vi "Host Image Acquisition Loop.vi"(8 "error in":errorcluster) -> (0 "error out":errorcluster)   [LabVIEW 2013]
doc: "Loop handles the image acquisition communication to FPGA.\nInitialize - Queues up the intialize states\n\nExit"
uses:
  Host Image Acquisition Module Enum.ctl
  Message Passing/MsgQ Loops enum.ctl
  File IO/Save Image Module Enum.ctl
  Image Acquisition Settings FG Enum.ctl
  System Status/Status FG Enum.ctl
  Globals/Simulation Settings Global.vi
  Common/State Machines/State Machine Lib.lvlib
  Message Passing/Main MsgQ.lvlib
panel:
  out "State":string
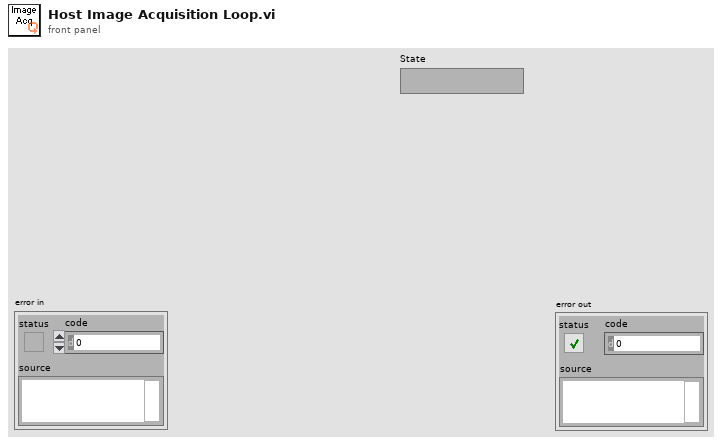
[diagram p1: front panel]
types:
  T1 = typedef "State Machine Lib.lvlib/STATE cluster.ctl" = cluster{"State":string, "Parameters":variant}
  T2 = typedef "Host Image Acquisition Module Enum.ctl" = enum16{"Open FPGA", "Initialize DMA FIFO", "Load Sim Images", "Initialize Acquisition", "Update Sector Parameters", "Start Acquisition", "Aquire Image", "Read Averages", "Cancel Acquisition", "Close FPGA"}
  T3 = typedef "Main MsgQ.lvlib/MsgQ Loops enum.ctl" = enum16{"User Interface", "Image Acq"}
  T4 = typedef "Save Image Module Enum.ctl" = enum16{"Create File", "Write to File", "Status", "Close File"}
  T5 = typedef "Image Acquisition Settings FG Enum.ctl" = enum16{"Read", "Write"}
  T6 = typedef "Status FG Enum.ctl" = enum16{"Reset", "Read", "Write"}
  T7 = typedef "Simulation Settings Cluster.ctl" = cluster{"Sim Enabled?":bool, "Sim Path":path}
  T8 = typedef "Acquisition Settings Cluster.ctl" = cluster{"Image Width":u32, "Image Height":u32, "Frames To Acquire":u32, "Signal Mapping":enum8{"Standard", "Basler 10-tap", "Vosskühler 10-tap"}, "DMA Buffer Size\n(In Images)":u32}
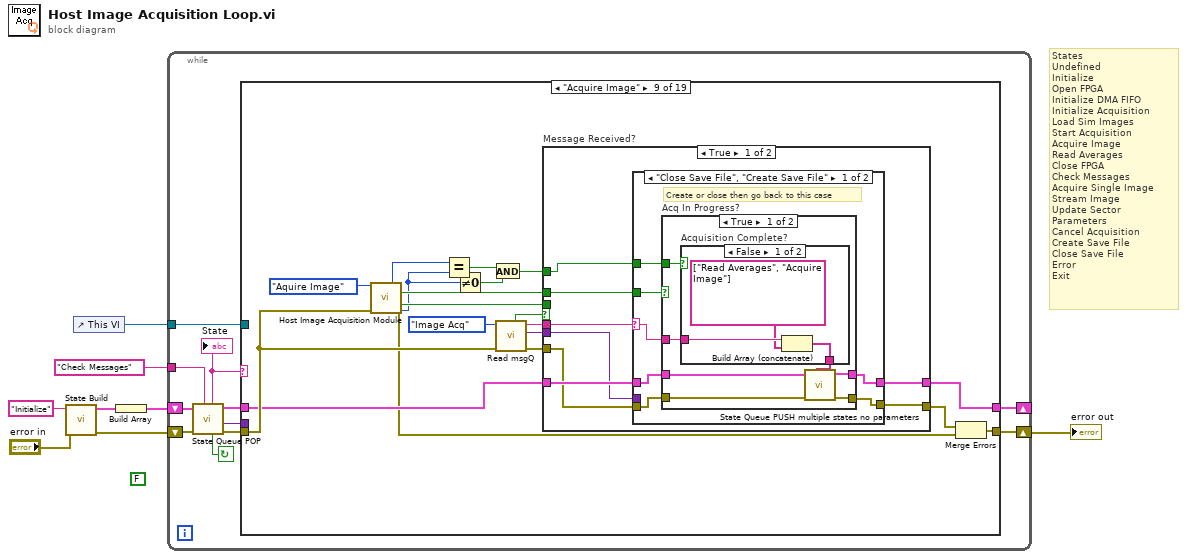
[diagram p0: block diagram]
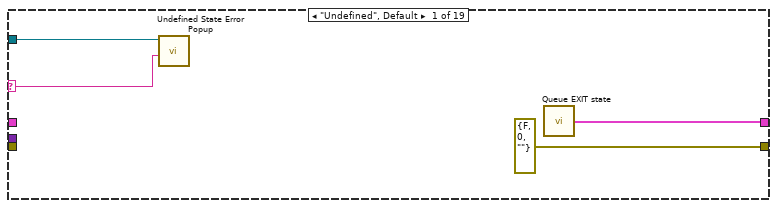
[diagram p2: hidden frame]
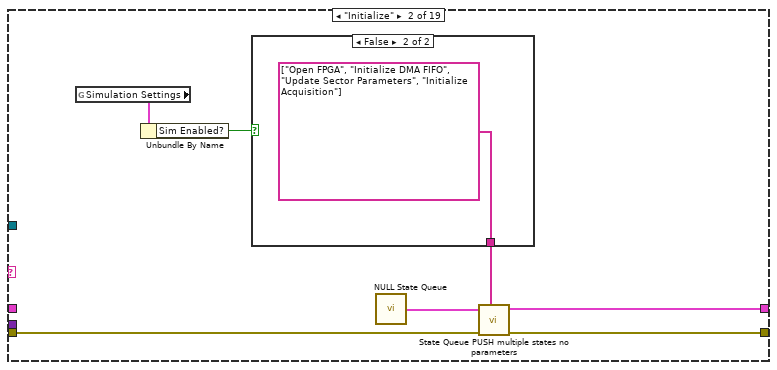
[diagram p3: hidden frame]
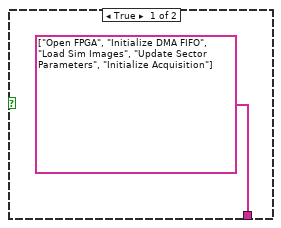
[diagram p4: hidden frame]
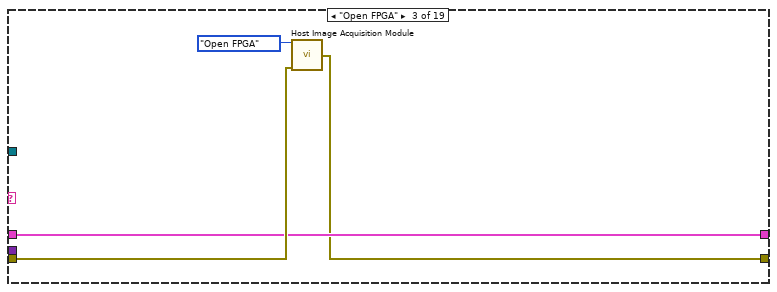
[diagram p5: hidden frame]
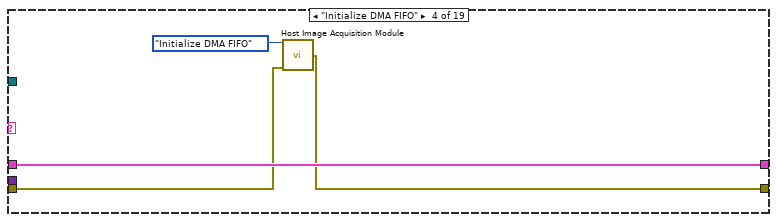
[diagram p6: hidden frame]
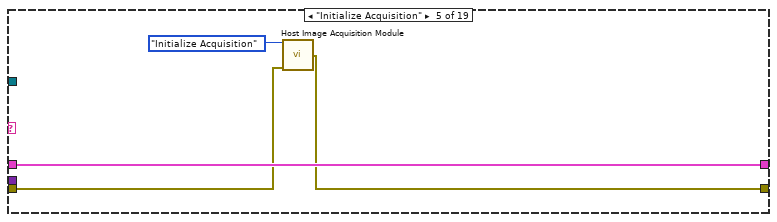
[diagram p7: hidden frame]
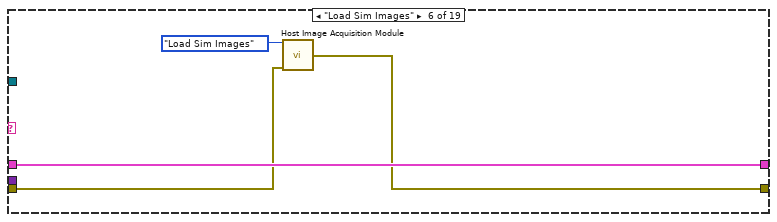
[diagram p8: hidden frame]
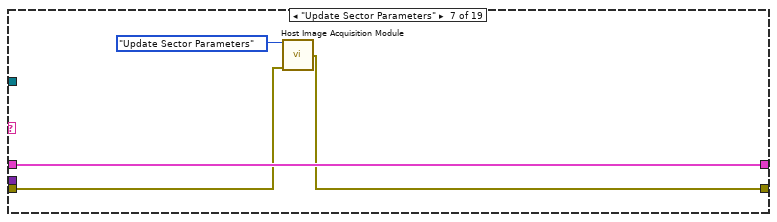
[diagram p9: hidden frame]
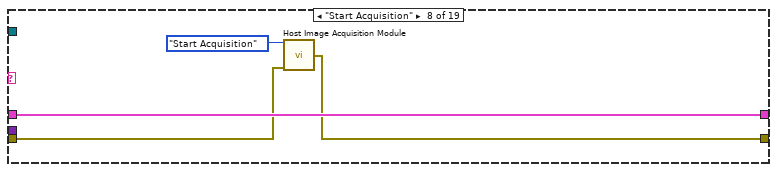
[diagram p10: hidden frame]
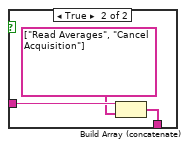
[diagram p11: hidden frame]
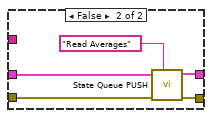
[diagram p12: hidden frame]
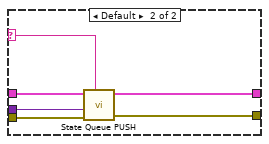
[diagram p13: hidden frame]
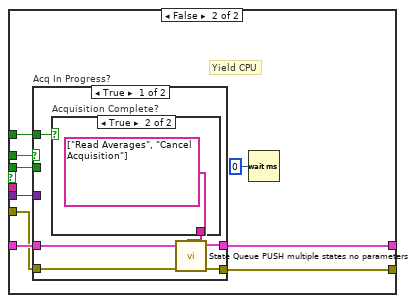
[diagram p14: hidden frame]
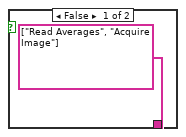
[diagram p15: hidden frame]
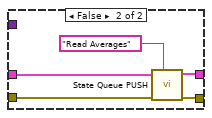
[diagram p16: hidden frame]
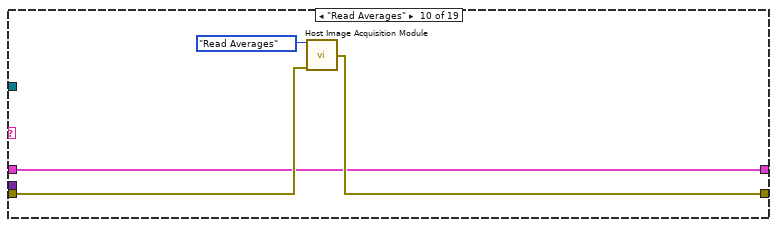
[diagram p17: hidden frame]
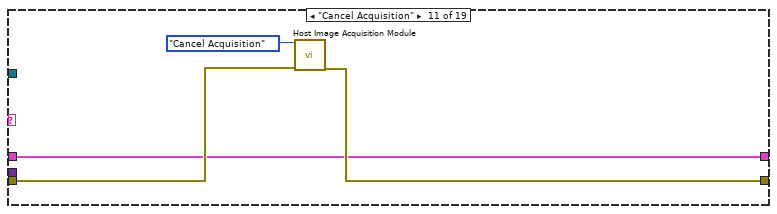
[diagram p18: hidden frame]
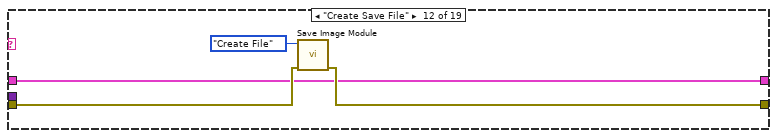
[diagram p19: hidden frame]
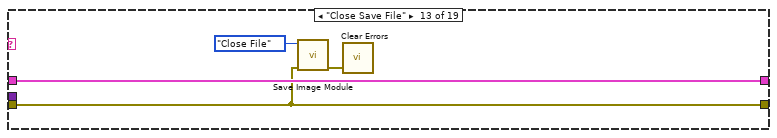
[diagram p20: hidden frame]
diagram:
  (unwired) FALSE
  # "States\nUndefined\nInitialize\nOpen FPGA\nInitialize DMA FIFO\nInitialize Acquisition\nLoad Sim Images\nStart Acquisition\nAcquire Image\nRead Averages\nClose FPGA\nCheck Messages\nAcquire Single Image\nStream Image\nUpdate Sector Parameters\nCancel Acquisition\nCreate Save File\nClose Save File\nError\nExit"
  n1 = call "State Build.vi"("error in (no error)"="error in", "State"="Initialize") -> ("error out"=w4:errorcluster, "State Out"=w6:T1)  [unwired: 8 in]
  n2 = control-ref of="This VI"() -> (w1:refnum<vi>)
  n3 = Build Array(w6) -> (w5:T1[])
  n4 = while {
    shift-right: [w12] -> _
    shift-left: w5 -> [w19]
    shift-right: [w11] -> w2
    shift-left: w4 -> [w18]
    tunnel: "Check Messages" ("Default state") -> [w16]
    tunnel: w1 -> [w10]
    stop <- w17 continue-if-true
    n5 = call "State Queue POP.vi"("Default state"=w16, "error in (no error)"=w18, "State que in"=w19) -> ("error out"=w13:errorcluster, "Parameters"=w9:variant, "State que out"=w14:T1[], "Not Exit?"=w17:bool, "State case out"=w15:string)  [unwired: 4 in]
    "State" <- w15
    n6 = case shown="\"Acquire Image\"" w15 {
      selector: w15 -> [w22 _ _ _ _ _ _ _ _ _ _ _ _ _ _ _ _ _ _]
      tunnel: w14 -> [_ _ w34 w40 w44 w48 w52 w56 w73 w137 w141 w145 w151 w156 w163 w178 w199 w219 w226]
      tunnel: w13 -> [_ w30 w35 w39 w43 w47 w51 w55 w74 w139 w143 w147 w149 w155 w165 w185 w189 w222 w225]
      tunnel: [w21 w27 w34 w40 w44 w48 w52 w56 w72 w137 w141 w145 w151 w156 w162 w176 w194 w219 w226] -> w12
      tunnel: [errorcluster {"status"=FALSE, "code"=0, "source"=""} ("error out") w26 w33 w38 w42 w45 w50 w54 w70 w138 w142 w146 w149 w154 w161 w175 w192 w220 w225] -> w11
      tunnel: w10 -> [w23 _ _ _ _ _ _ _ _ _ _ _ _ _ _ _ _ _ _]
      tunnel: w9 -> [_ _ _ _ _ _ _ _ _ _ _ _ _ _ _ _ w198 _ _]
      frame "Undefined", Default {
        n7 = call "Undefined State Error Popup.vi"("String"=w22, "This VI (Caller if unwired)"=w23) -> ()  [unwired: 10 in]
        n8 = call "Queue EXIT state.vi"() -> ("Exit State Q"=w21:T1[])  [unwired: 1 in]
      }
      frame "Initialize" {
        n9 = global read "Simulation Settings Global.vi" "Simulation Settings"() -> (w25:T7)
        n10 = Unbundle By Name(w25) -> ("Sim Enabled?"=w24:bool)
        n11 = case shown="False" w24 {
          tunnel: [string[] ["Open FPGA", "Initialize DMA FIFO", "Load Sim Images", "Update Sector Parameters", "Initialize Acquisition"] ("States to queue") string[] ["Open FPGA", "Initialize DMA FIFO", "Update Sector Parameters", "Initialize Acquisition"] ("States to queue")] -> w28
          frame True {
          }
          frame False {
          }
        }
        n12 = call "NULL State Queue.vi"() -> ("NULL State Queue"=w29:T1[])
        n13 = call "State Queue PUSH multiple states no parameters.vi"("States to queue"=w28, "error in (no error)"=w30, "State que in"=w29) -> ("error out"=w26:errorcluster, "State que out"=w27:T1[])  [unwired: 7 in]
      }
      frame "Open FPGA" {
        n14 = call "Host Image Acquisition Module.vi"("Operation"=Host_Image_Acquisition_Module_Enum."Open FPGA", "error in"=w35) -> ("error out"=w33:errorcluster)  [unwired: 6 in, 7 out]
      }
      frame "Initialize DMA FIFO" {
        n15 = call "Host Image Acquisition Module.vi"("Operation"=Host_Image_Acquisition_Module_Enum."Initialize DMA FIFO", "error in"=w39) -> ("error out"=w38:errorcluster)  [unwired: 6 in, 7 out]
      }
      frame "Initialize Acquisition" {
        n16 = call "Host Image Acquisition Module.vi"("Operation"=Host_Image_Acquisition_Module_Enum."Initialize Acquisition", "error in"=w43) -> ("error out"=w42:errorcluster)  [unwired: 6 in, 7 out]
      }
      frame "Load Sim Images" {
        n17 = call "Host Image Acquisition Module.vi"("Operation"=Host_Image_Acquisition_Module_Enum."Load Sim Images", "error in"=w47) -> ("error out"=w45:errorcluster)  [unwired: 6 in, 7 out]
      }
      frame "Update Sector Parameters" {
        n18 = call "Host Image Acquisition Module.vi"("Operation"=Host_Image_Acquisition_Module_Enum."Update Sector Parameters", "error in"=w51) -> ("error out"=w50:errorcluster)  [unwired: 6 in, 7 out]
      }
      frame "Start Acquisition" {
        n19 = call "Host Image Acquisition Module.vi"("Operation"=Host_Image_Acquisition_Module_Enum."Start Acquisition", "error in"=w55) -> ("error out"=w54:errorcluster)  [unwired: 6 in, 7 out]
      }
      frame "Acquire Image" {
        n20 = call "Host Image Acquisition Module.vi"("Operation"=Host_Image_Acquisition_Module_Enum."Aquire Image", "error in"=w74) -> ("Num Frames read"=w61:u32, "Acq In Progress"=w69:bool, "error out"=w71:errorcluster, "Image Acquired"=w68:bool, "Frames To Acquire"=w57:u32)  [unwired: 6 in, 3 out]
        n21 = Equal?(x=w61, y=w57) -> (x = y?=w60:bool)
        n22 = Not Equal To 0?(x=w57) -> (x != 0?=w58:bool)
        n23 = And(x=w60, y=w58) -> (x .and. y?=w59:bool)
        n24 = call "Read msgQ.vi"("error in"=w74, "MsgQ enum"=MsgQ_Loops_enum."Image Acq") -> ("error out"=w64:errorcluster, "Message Received Parameters"=w62:variant, "Message Received String"=w65:string, "Message Recieved?"=w66:bool)  [unwired: 6 in]
        n25 = case "Message Received?" shown="True" w66 {
          tunnel: w65 -> [w78 _]
          tunnel: w64 -> [w82 w122]
          tunnel: w73 -> [w83 w123]
          tunnel: [w81 w121] -> w63
          tunnel: [w80 w120] -> w72
          tunnel: w69 -> [w77 w119]
          tunnel: w62 -> [w79 w118]
          tunnel: w68 -> [_ w117]
          tunnel: w59 -> [w76 w116]
          frame True {
            n26 = case shown="\"Close Save File\", \"Create Save File\"" w78 {
              selector: w78 -> [w87 w109]
              tunnel: w83 -> [w89 w114]
              tunnel: w82 -> [w88 w113]
              tunnel: [w84 w112] -> w81
              tunnel: [w85 w111] -> w80
              tunnel: w79 -> [_ w110]
              tunnel: w77 -> [w90 _]
              tunnel: w76 -> [w86 _]
              frame "Close Save File", "Create Save File" {
                # "Create or close then go back to this case"
                n27 = case "Acq In Progress?" shown="True" w90 {
                  tunnel: w89 -> [w97 w108]
                  tunnel: w88 -> [w94 w105]
                  tunnel: [w95 w106] -> w84
                  tunnel: [w96 w107] -> w85
                  tunnel: w86 -> [w92 _]
                  tunnel: w87 -> [w91 _]
                  frame True {
                    n28 = case "Acquisition Complete?" shown="False" w92 {
                      tunnel: [w98 w101] -> w93
                      tunnel: w91 -> [w100 w103]
                      frame False {
                        n29 = Build Array (concatenate)(w100, string[] ["Read Averages", "Acquire Image"] ("States to queue")) -> (w98:string[])
                      }
                      frame True {
                        n30 = Build Array (concatenate)(w103, string[] ["Read Averages", "Cancel Acquisition"] ("States to queue")) -> (w101:string[])
                      }
                    }
                    n31 = call "State Queue PUSH multiple states no parameters.vi"("States to queue"=w93, "error in (no error)"=w94, "State que in"=w97) -> ("error out"=w95:errorcluster, "State que out"=w96:T1[])  [unwired: 7 in]
                  }
                  frame False {
                    n32 = call "State Queue PUSH.vi"("State case"="Read Averages", "error in (no error)"=w105, "State que in"=w108) -> ("error out"=w106:errorcluster, "State que out"=w107:T1[])  [unwired: 7 in]
                  }
                }
              }
              frame Default {
                n33 = call "State Queue PUSH.vi"("State case"=w109, "error in (no error)"=w113, "Parameters"=w110, "State que in"=w114) -> ("error out"=w112:errorcluster, "State que out"=w111:T1[])  [unwired: 6 in]
              }
            }
          }
          frame False {
            # "Yield CPU"
            n34 = case "Acq In Progress?" shown="True" w119 {
              tunnel: w123 -> [w129 w136]
              tunnel: w122 -> [w126 w133]
              tunnel: [w127 w134] -> w121
              tunnel: [w128 w135] -> w120
              tunnel: w118 -> [_ _]
              tunnel: w117 -> [_ _]
              tunnel: w116 -> [w124 _]
              frame True {
                n35 = case "Acquisition Complete?" shown="True" w124 {
                  tunnel: [string[] ["Read Averages", "Acquire Image"] ("States to queue") string[] ["Read Averages", "Cancel Acquisition"] ("States to queue")] -> w125
                  frame False {
                  }
                  frame True {
                  }
                }
                n36 = call "State Queue PUSH multiple states no parameters.vi"("States to queue"=w125, "error in (no error)"=w126, "State que in"=w129) -> ("error out"=w127:errorcluster, "State que out"=w128:T1[])  [unwired: 7 in]
              }
              frame False {
                n37 = call "State Queue PUSH.vi"("State case"="Read Averages", "error in (no error)"=w133, "State que in"=w136) -> ("error out"=w134:errorcluster, "State que out"=w135:T1[])  [unwired: 7 in]
              }
            }
            n38 = Wait (ms)(milliseconds to wait=u32 0) -> ()  [unwired: 1 out]
          }
        }
        n39 = Merge Errors(w63, w71) -> (w70:errorcluster)
      }
      frame "Read Averages" {
        n40 = call "Host Image Acquisition Module.vi"("Operation"=Host_Image_Acquisition_Module_Enum."Read Averages", "error in"=w139) -> ("error out"=w138:errorcluster)  [unwired: 6 in, 7 out]
      }
      frame "Cancel Acquisition" {
        n41 = call "Host Image Acquisition Module.vi"("Operation"=Host_Image_Acquisition_Module_Enum."Cancel Acquisition", "error in"=w143) -> ("error out"=w142:errorcluster)  [unwired: 6 in, 7 out]
      }
      frame "Create Save File" {
        n42 = call "Save Image Module.vi"("error in"=w147, "Mode"=Save_Image_Module_Enum."Create File") -> ("error out"=w146:errorcluster)  [unwired: 8 in, 1 out]
      }
      frame "Close Save File" {
        n43 = call "Save Image Module.vi"("error in"=w149, "Mode"=Save_Image_Module_Enum."Close File") -> ("error out"=w150:errorcluster)  [unwired: 8 in, 1 out]
        n44 = call <vilib>:"Clear Errors.vi"("error in (no error)"=w150) -> ()  [unwired: 6 in, 1 out]
      }
      frame "Close FPGA" {
        n45 = call "Host Image Acquisition Module.vi"("Operation"=Host_Image_Acquisition_Module_Enum."Close FPGA", "error in"=w155) -> ("error out"=w154:errorcluster)  [unwired: 6 in, 7 out]
      }
      frame "Check Messages" {
        n46 = call "Read msgQ.vi"("error in"=w165, "MsgQ enum"=MsgQ_Loops_enum."Image Acq") -> ("error out"=w160:errorcluster, "Message Received Parameters"=w157:variant, "Message Received String"=w159:string, "Message Recieved?"=w164:bool)  [unwired: 6 in]
        n47 = case shown="True" w164 {
          tunnel: w163 -> [w168 w174]
          tunnel: [w168 w173] -> w162
          tunnel: [w167 w172] -> w161
          tunnel: w160 -> [w167 w171]
          tunnel: w159 -> [_ w169]
          tunnel: w157 -> [_ w170]
          frame False {
            # "Yield CPU"
            n48 = Wait (ms)(milliseconds to wait=u32 0) -> ()  [unwired: 1 out]
          }
          frame True {
            n49 = call "State Queue PUSH.vi"("State case"=w169, "error in (no error)"=w171, "Parameters"=w170, "State que in"=w174) -> ("error out"=w172:errorcluster, "State que out"=w173:T1[])  [unwired: 6 in]
          }
        }
      }
      frame "Acquire Single Image" {
        n50 = call "Image Acquisition Settings FG.vi"("error in (no error)"=w185, "Operation"=Image_Acquisition_Settings_FG_Enum."Read") -> ("error out"=w180:errorcluster, "Acquisition Settings Out"=w184:T8)  [unwired: 8 in]
        n51 = Bundle By Name(cluster=w184, "Frames To Acquire"=u32 1) -> (w182:T8)
        n52 = call "Image Acquisition Settings FG.vi"("error in (no error)"=w180, "Acquisition Settings In"=w182, "Operation"=Image_Acquisition_Settings_FG_Enum."Write") -> ("error out"=w179:errorcluster)  [unwired: 7 in, 1 out]
        n53 = call "State Queue PUSH multiple states no parameters.vi"("States to queue"=string[] ["Start Acquisition", "Acquire Image"], "error in (no error)"=w179, "State que in"=w178) -> ("error out"=w175:errorcluster, "State que out"=w176:T1[])  [unwired: 7 in]
      }
      frame "Stream Image" {
        n54 = global read "Simulation Settings Global.vi" "Simulation Settings"() -> (w190:T7)
        n55 = Unbundle By Name(w190) -> ("Sim Enabled?"=w187:bool)
        n56 = Variant To Data(error in=w189, type=TRUE, Variant=w198) -> (data=w196:bool, error out=w188:errorcluster)
        n57 = case "Enable Stream?" shown="True" w196 {
          tunnel: w188 -> [w200 w207]
          tunnel: w199 -> [w201 w206]
          tunnel: [w201 w206] -> w195
          tunnel: [w200 w205] -> w193
          tunnel: [string[] ["Cancel Acquisition", "Close Save File"] ("States to queue") string[] ["Start Acquisition", "Acquire Image"] ("States to queue")] -> w191
          tunnel: w187 -> [_ w203]
          frame False {
          }
          frame True {
            n58 = case shown="False" w203 {
              tunnel: w207 -> [w214 w216]
              tunnel: [w208 w216] -> w205
              frame False {
                n59 = call "Image Acquisition Settings FG.vi"("error in (no error)"=w214, "Operation"=Image_Acquisition_Settings_FG_Enum."Read") -> ("error out"=w209:errorcluster, "Acquisition Settings Out"=w213:T8)  [unwired: 8 in]
                n60 = Bundle By Name(cluster=w213, "Frames To Acquire"=u32 0) -> (w211:T8)
                n61 = call "Image Acquisition Settings FG.vi"("error in (no error)"=w209, "Acquisition Settings In"=w211, "Operation"=Image_Acquisition_Settings_FG_Enum."Write") -> ("error out"=w208:errorcluster)  [unwired: 7 in, 1 out]
              }
              frame True {
              }
            }
          }
        }
        n62 = call "State Queue PUSH multiple states no parameters.vi"("States to queue"=w191, "error in (no error)"=w193, "State que in"=w195) -> ("error out"=w192:errorcluster, "State que out"=w194:T1[])  [unwired: 7 in]
      }
      frame "Error" {
        n63 = Unbundle By Name(w222) -> ("source"=w223:string)
        n64 = Concatenate Strings("Error: " ("string"), w223) -> (w218:string)
        n65 = call "Status FG.vi"("Status In"=w218, "Operation"=Status_FG_Enum."Write") -> ()  [unwired: 8 in, 2 out]
        n66 = call "Broadcast Exit.vi"("error in"=errorcluster {"status"=FALSE, "code"=0, "source"=""}) -> ("error out"=w220:errorcluster)  [unwired: 10 in]
      }
      frame "Exit" {
      }
    }
  }
  "error out" <- w2
